vi "Callback Change Tag.vi"(6 "Variant":variant, 8 "error in (no error)":errorcluster, 9 "Old Values":string[][](array[string]), 10 "object ref in":T1, 11 "Table Change":T2) -> (0 "error out":errorcluster)   [LabVIEW 2015, in "SystemLink File editor node.lvclass"]
doc: "This VI gets called automatically when changes are made to the 'Tag' column of the table and must handle changes appropriately. Register this callback using the appropriate 'Define Column' VI from the Table API."
uses:
  SystemLink File editor node.lvclass
  <vilib>/NI/DCAF/Tag Editor Core/Table API/Table Manager/Cell Change.ctl
  <vilib>/NI/DCAF/Tag Editor Core/Table API/Table Manager/object ref.ctl
  <vilib>/NI/DCAF/Tag Editor Core/Configuration Editor/Classes/Engine Parent/Engine Parent Editor Node.lvclass
  <vilib>/NI/DCAF/Tag Editor Core/Configuration Editor/Classes/Module editor node/module editor node.lvclass
  <vilib>/NI/Tag Bus Module Framework/channel/TBM channel.lvclass
  module/configuration/SystemLink File configuration.lvclass
  <vilib>/NI/DCAF/Tag Editor Core/Table API/Table Manager.lvlib
  <vilib>/NI/DCAF/Tag Editor Core/Table API/Table Manager/Table Manager.lvclass
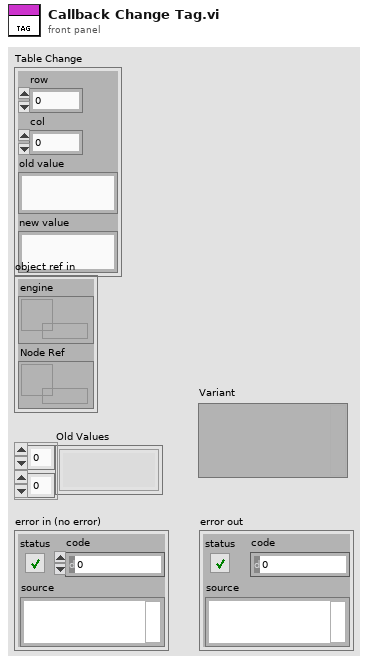
[diagram p1: front panel]
types:
  T1 = typedef "Table Manager.lvlib/Table Manager.lvclass/object ref.ctl" = cluster{"engine":refnum<data-value>, "Node Ref":refnum<data-value>}
  T2 = typedef "Table Manager.lvlib/Cell Change.ctl" = cluster{"row":i32, "col":i32, "old value":string, "new value":string}
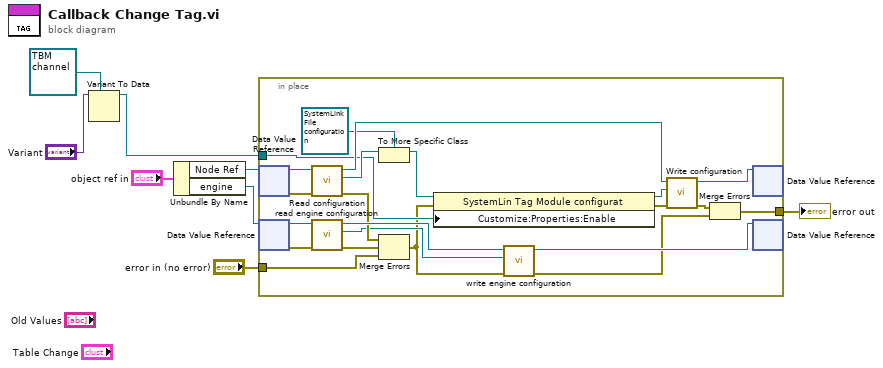
[diagram p0: block diagram]
diagram:
  n1 = Variant To Data(type=refnum<class "TBM channel.lvclass"> refnum ("output"), Variant="Variant") -> (data=w1:refnum<class "TBM channel.lvclass">)  [unwired: 1 in, 1 out]
  n2 = Unbundle By Name("object ref in") -> ("Node Ref"=w5:refnum<data-value>, "engine"=w4:refnum<data-value>)
  n3 = in-place {
    in-place-border: [w22] -> w8
    in-place-border: "error in (no error)" -> [w16]
    in-place-border: w1 -> [w12]
    n4 = in-place-dvr #1(w5) -> (w19:refnum<class "module editor node.lvclass">, w21:errorcluster)
    n5 = in-place-dvr #2(w4) -> (w29:refnum<class "Engine Parent Editor Node.lvclass">, w30:errorcluster)
    n6 = call-dynamic "Read configuration.vi"("error in"=w21, "NISE_CEF_serializable node in"=w19) -> ("error out"=w20:errorcluster, "configuration"=w17:refnum<class "NISE_CEF_serializable configuration.lvclass">, "NISE_CEF_serializable node out"=w18:refnum<class "module editor node.lvclass">)  [unwired: 7 in]
    n7 = call <vilib>:"read engine configuration.vi"("error in"=w30, "Engine Parent Editor Node in"=w29) -> ("error out"=w26:errorcluster, "engine configuration"=w15:refnum<class "engine configuration.lvclass">, "Engine Parent Editor Node out"=w25:refnum<class "Engine Parent Editor Node.lvclass">)  [unwired: 7 in]
    n8 = To More Specific Class(target class=refnum<class "SystemLink File configuration.lvclass"> refnum ("tag bus configurable plugin module configuration"), reference=w17) -> (specific class reference=w13:refnum<class "SystemLink File configuration.lvclass">)  [unwired: 1 in, 1 out]
    n9 = Merge Errors(w20, w26, w16) -> (w10:errorcluster)
    n10 = property class="SystemLin Tag Module configurat"(reference=w13, error in=w10, "Customize:Properties:Enable"=w12) -> (reference out=w11:refnum<class "SystemLink File configuration.lvclass">, error out=w9:errorcluster)
    n11 = call <vilib>:"write engine configuration.vi"("error in"=w10, "engine configuration"=w15, "Engine Parent Editor Node in"=w25) -> ("error out"=w24:errorcluster, "Engine Parent Editor Node out"=w28:refnum<class "Engine Parent Editor Node.lvclass">)  [unwired: 7 in]
    n12 = call-dynamic "Write configuration.vi"("error in"=w9, "configuration"=w11, "NISE_CEF_serializable node in"=w18) -> ("error out"=w23:errorcluster, "NISE_CEF_serializable node out"=w27:refnum<class "module editor node.lvclass">)  [unwired: 7 in]
    n13 = Merge Errors(w23, w24) -> (w22:errorcluster)
    n14 = in-place-dvr #1(w27) -> ()  [unwired: 2 out]
    n15 = in-place-dvr #2(w28) -> ()  [unwired: 2 out]
  }
  "error out" <- w8
